vi "OnCFXMessageReceivedFromListener.vi"(4 "FromListener":refnum<vi>, 5 "事件数据":T1, 6 "控件引用":refnum<k24>, 7 "事件通用数据":cluster{"事件源":i32, "事件类型":u32, "时间标识":u32}) -> ()   [LabVIEW 2025]
uses:
  CFX_dll/CFX.dll
panel:
  out "错误输出":errorcluster
  in  "错误输入（无错误）":errorcluster
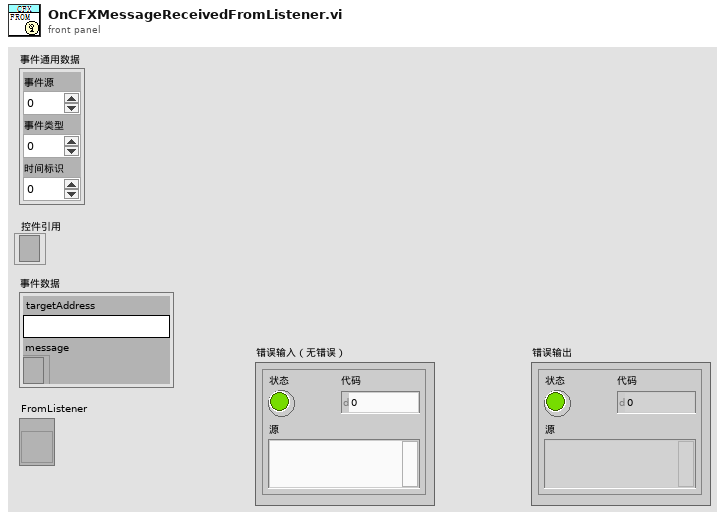
[diagram p1: front panel]
types:
  T1 = cluster{"targetAddress":string, "message":refnum<k24>}
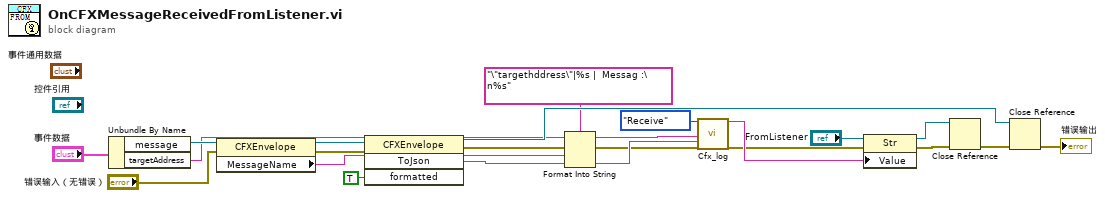
[diagram p0: block diagram]
diagram:
  n1 = Unbundle By Name("事件数据") -> ("message"=w17:refnum<k24>, "targetAddress"=w8:string)
  n2 = property on="属性节点" class="CFXEnvelope"(reference=w17, error in="错误输入（无错误）") -> (reference out=w12:refnum<k24>, error out=w3:errorcluster, "MessageName"=w7:string)
  n3 = invoke class="CFXEnvelope" method="ToJson"(reference=w12, error in=w3, "formatted"=TRUE) -> (reference out=w16:refnum<k24>, error out=w2:errorcluster, "ToJson"=w4:string)  [unwired: 1 in, 1 out]
  n4 = Format Into String(format string="\"targethddress\"|%s |  Messag :\n%s" ("格式字符串"), initial string=w8, error in=w2, w7, w4) -> (resulting string=w9:string, error out=w1:errorcluster)
  n5 = call "Cfx_log.vi"("R/W"=enum16{"Send", "Receive"}."Receive", "Message_Name"=w9, "Message_Content"=w4, "error in"=w1) -> ("Log_out"=w11:string, "error out"=w10:errorcluster)  [unwired: 14 in]
  n6 = property on="属性节点" class="Str"(reference="FromListener", error in=w10, "Value"=w11) -> (reference out=w19:refnum<vi>, error out=w18:errorcluster)
  n7 = Close Reference(reference=w19, error in (no error)=w18) -> (error out=w14:errorcluster)
  n8 = Close Reference(reference=w16, error in (no error)=w14) -> (error out=→"错误输出":errorcluster)
